vi "VIH HelpGen - Write HTML File - VI.vi"(6 "Owning Palette":cluster{"Name":string, "HTML Path":path}, 8 "error in":errorcluster, 9 "HTML Path":path, 10 "VI Path":path, 11 "Project Tree":T1) -> (0 "error out":errorcluster, 3 "dup Project Tree":T1)   [LabVIEW 2014]
doc: "::: VI Helpeks :::\nCopyright (c) 2000-2026 Konstantin Shifershteyn. All rights reserved."
uses:
  _VIH Project Manager.llb/VIH Project Tree Typedef - Tree Refnum.ctl
panel:
  # "VI Helpeks\nCopyright (c) 2012-2026 Konstantin Shifershteyn"
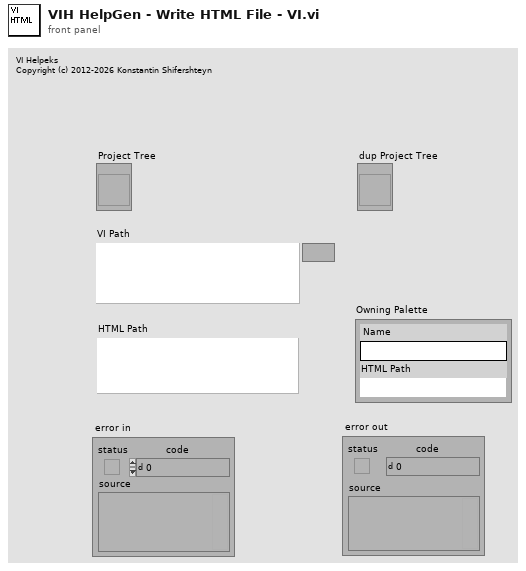
[diagram p1: front panel]
types:
  T1 = typedef "VIH Project Tree Typedef - Tree Refnum.ctl" = refnum<vi>
  T2 = typedef "VIH HelpGen Typedef - Cluster - File Rule.ctl" = cluster{"OutName":string, "BuildHelp":T3, "Source Paths":T4, "Target Paths":T5, "DscrMode":T6, "Description":string, "Control Rules":T7[], "Flags":T9, "Ctl_DscrMode":T6, "Ctl_ClustMembers":T3, "Ctl_EnumValues":T3, "MenuItemIcons":T3, "%Comments":string, "DetailsMode":T6, "DetailsText":string, "ProductInfoMode":T3, "ProductInfoText":string}
  T3 = typedef "VIH HelpGen Typedef - Enum - Default,Enable,Disable.ctl" = enum16{"Default", "Enable", "Disable"}
  T4 = typedef "VIH HelpGen Typedef - Cluster - File Rule - Source Paths.ctl" = cluster{"CSS Files":path[], "JS Files":path[], "Html Template":path}
  T5 = typedef "VIH HelpGen Typedef - Cluster - File Rule - Target Paths.ctl" = cluster{"HTML Dir":path, "Image Dir":path, "CSS Dir":path, "JS Dir":path}
  T6 = typedef "VIH HelpGen Typedef - Enum - Description Mode.ctl" = enum16{"Default", "Description", "Description1", "Description2", "Custom", "None"}
  T7 = typedef "VIH HelpGen Typedef - Cluster - Control Rule.ctl" = cluster{"CtrlID":string, "CustomRule":bool, "DscrMode":T6, "Description":string, "ClusterMembers":T3, "EnumValues":T3, "EnumValDscr":T8[], "CustomName":string}
  T8 = typedef "VIH HelpGen Typedef - Cluster - Enum Value Info.ctl" = cluster{"Value":ext, "String":string, "Description":string}
  T9 = typedef "VIH HelpGen Typedef - Cluster - Group Rule - Flags.ctl" = cluster{"Override CSS Files":bool, "Override JS Files":bool, "Override Ctl Rules":bool}
  T10 = typedef "imagedata.ctl" = cluster{"image type":i32, "image depth":i32, "image":u8[], "mask":u8[], "colors":u32[], "Rectangle":cluster{"left":i16, "top":i16, "right":i16, "bottom":i16}}
  T11 = cluster{"Original VI Name":string, "Conpane Image":T10}
  T12 = cluster{"ProductInfoMode":T3, "ProductInfoText":string}
  T13 = typedef "VIH HelpGen Typedef - Table Templates Cluster - VI Help.ctl" = cluster{"Ctrl Dscr":string, "Ring Val Dscr":string, "Enum Val Dscr":string, "VI Details":string}
  T14 = cluster{"directory path out":path, "directory path out":path, "name":string}
  T15 = cluster{string[], "Control Rules":T7[], "Ctl_DscrMode":T6, "Ctl_ClustMembers":T3, "Ctl_EnumValues":T3}
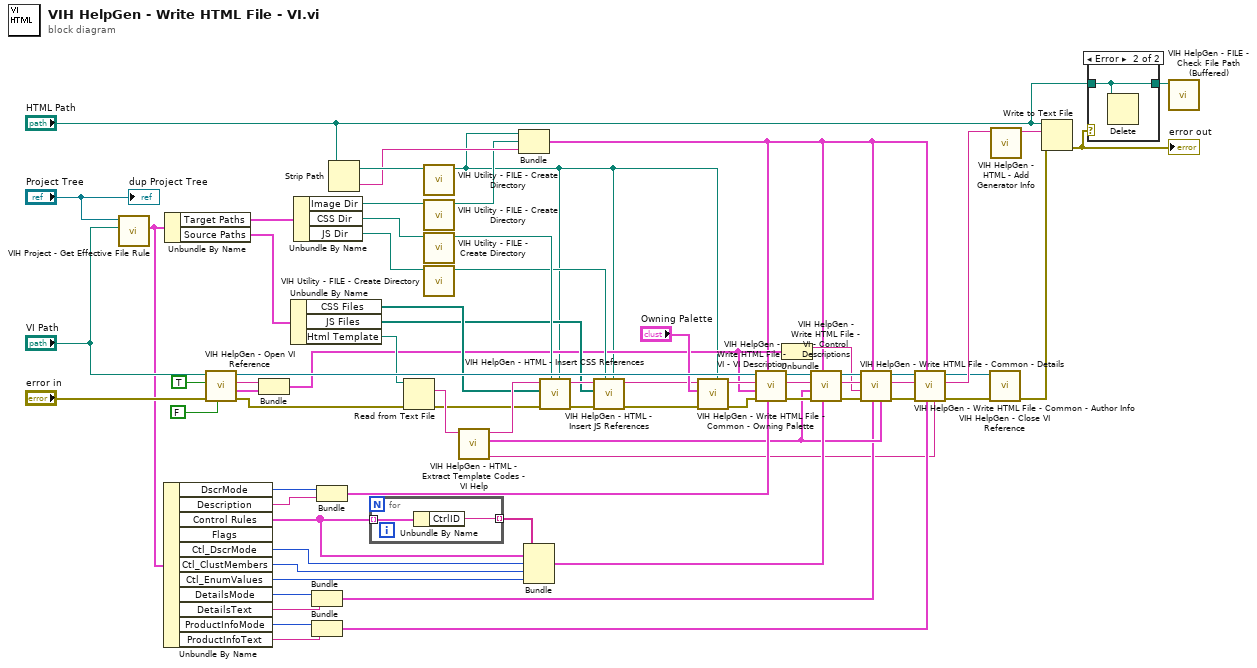
[diagram p0: block diagram]
diagram:
  n1 = call "VIH Project - Get Effective File Rule.vi"("File Path"="VI Path", "Project Tree"="Project Tree") -> ("Effective File Rule"=w48:T2)  [unwired: 6 in, 3 out]
  n2 = Unbundle By Name(w48) -> ("DscrMode"=w47:T6, "Description"=w46:string, "Control Rules"=w41:T7[], "Ctl_DscrMode"=w44:T6, "Ctl_ClustMembers"=w43:T3, "Ctl_EnumValues"=w42:T3, "DetailsMode"=w27:T6, "DetailsText"=w26:string, "ProductInfoMode"=w9:T3, "ProductInfoText"=w8:string)  [unwired: 1 out]
  n3 = Unbundle By Name(w48) -> ("Target Paths"=w63:T5, "Source Paths"=w62:T4)
  n4 = call "VIH HelpGen - Open VI Reference.vi"("Enable Conpane Image Check (T)"=FALSE, "error in"="error in", "Force use wrapper (F)"=TRUE, "VI Path"="VI Path") -> ("error out"=w59:errorcluster, "Conpane Image"=w22:T10, "Original VI Name"=w23:string, "VI Reference"=w65:refnum<vi>)  [unwired: 4 in]
  n5 = Bundle("Original VI Name"=w23, "Conpane Image"=w22) -> (w21:T11)  [unwired: 1 in]
  n6 = Unbundle By Name(w62) -> ("CSS Files"=w61:path[], "JS Files"=w32:path[], "Html Template"=w60:path)
  n7 = Unbundle By Name(w63) -> ("Image Dir"=w49:path, "CSS Dir"=w51:path, "JS Dir"=w38:path)
  n8 = Bundle("DetailsMode"=w27, "DetailsText"=w26) -> (w24:cluster{"DetailsMode":T6, "DetailsText":string})  [unwired: 1 in]
  n9 = Bundle("ProductInfoMode"=w9, "ProductInfoText"=w8) -> (w7:T12)  [unwired: 1 in]
  n10 = Bundle("DscrMode"=w47, "Description"=w46) -> (w45:cluster{"DscrMode":T6, "Description":string})  [unwired: 1 in]
  n11 = Strip Path(path="HTML Path") -> (stripped path=w52:path, name=w4:string)
  n12 = for {
    tunnel: w41 -> [w73] mode=indexing
    tunnel: [w72] -> w40 mode=indexing
    n13 = Unbundle By Name(w73) -> ("CtrlID"=w72:string)
  }
  n14 = Read from Text File(file (use dialog)=w60, error in=w59) -> (text=w67:string, error out=w58:errorcluster)  [unwired: 2 in, 2 out]
  n15 = call "VIH Utility - FILE - Create Directory.vi"("directory path"=w52) -> ("directory path out"=w1:path)  [unwired: 6 in, 2 out]
  n16 = call "VIH Utility - FILE - Create Directory.vi"("directory path"=w49) -> ("directory path out"=w3:path)  [unwired: 6 in, 2 out]
  n17 = call "VIH Utility - FILE - Create Directory.vi"("directory path"=w51) -> ("directory path out"=w50:path)  [unwired: 6 in, 2 out]
  n18 = call "VIH Utility - FILE - Create Directory.vi"("directory path"=w38) -> ("directory path out"=w33:path)  [unwired: 6 in, 2 out]
  n19 = call "VIH HelpGen - HTML - Extract Template Codes - VI Help.vi"("HTML in"=w67) -> ("ProductInfo Template"=w6:string, "Table Templates"=w25:T13, "HTML out"=w64:string)  [unwired: 8 in]
  n20 = Bundle("directory path out"=w1, "directory path out"=w3, "name"=w4) -> (w2:T14)  [unwired: 1 in]
  n21 = Bundle(w40, "Control Rules"=w41, "Ctl_DscrMode"=w44, "Ctl_ClustMembers"=w43, "Ctl_EnumValues"=w42) -> (w39:T15)  [unwired: 1 in]
  n22 = call "VIH HelpGen - HTML - Insert CSS References.vi"("HTML Folder"=w1, "CSS Folder"=w50, "error in"=w58, "CSS files"=w61, "HTML in"=w64) -> ("error out"=w36:errorcluster, "HTML out"=w37:string)  [unwired: 5 in]
  n23 = call "VIH HelpGen - HTML - Insert JS References.vi"("HTML Folder"=w1, "JSS Folder"=w33, "error in"=w36, "JS files"=w32, "HTML in"=w37) -> ("error out"=w35:errorcluster, "HTML out"=w34:string)  [unwired: 5 in]
  n24 = call "VIH HelpGen - Write HTML File - Common - Owning Palette.vi"("HTML Folder"=w1, "error in"=w35, "Owning Palette"="Owning Palette", "HTML in"=w34) -> ("error out"=w56:errorcluster, "HTML out"=w57:string)  [unwired: 6 in]
  n25 = call "VIH HelpGen - Write HTML File - VI - VI Description.vi"("Description Params"=w45, "Save params"=w2, "error in"=w56, "Original VI Info"=w21, "HTML in"=w57, "VI Reference"=w65) -> ("error out"=w69:errorcluster, "HTML out"=w68:string, "dup VI Reference"=w70:refnum<vi>)  [unwired: 3 in]
  n26 = Unbundle(w21) -> ("Original VI Name"=w20:string)  [unwired: 1 out]
  n27 = call "VIH HelpGen - Write HTML File - VI - Control Descriptions.vi"("Ctrl Dscr Params"=w39, "Save params"=w2, "error in"=w69, "Table Templates"=w25, "HTML in"=w68, "VI Reference"=w70) -> ("error out"=w28:errorcluster, "HTML out"=w29:string, "dup VI Reference"=w30:refnum<vi>)  [unwired: 3 in]
  n28 = call "VIH HelpGen - Write HTML File - Common - Details.vi"("Templates"=w25, "Details Params"=w24, "Save params"=w2, "error in"=w28, "Original VI Name"=w20, "HTML in"=w29, "VI Reference"=w30) -> ("error out"=w14:errorcluster, "HTML out"=w13:string, "dup VI Reference"=w15:refnum<vi>)  [unwired: 2 in]
  n29 = call "VIH HelpGen - Write HTML File - Common - Author Info.vi"("Product Info Template"=w6, "Product Info"=w7, "Save params"=w2, "error in"=w14, "HTML in"=w13, "VI Reference"=w15) -> ("error out"=w10:errorcluster, "HTML out"=w12:string, "dup VI Reference"=w11:refnum<vi>)  [unwired: 3 in]
  n30 = call "VIH HelpGen - Close VI Reference.vi"("error in"=w10, "VI Reference"=w11) -> ("error out"=w66:errorcluster)  [unwired: 9 in]
  n31 = call "VIH HelpGen - HTML - Add Generator Info.vi"("HTML in"=w12) -> ("HTML out"=w16:string)  [unwired: 10 in]
  n32 = Write to Text File(file (use dialog)="HTML Path", text=w16, error in=w66) -> (error out=w18:errorcluster)  [unwired: 1 in, 2 out]
  "error out" <- w18
  n33 = case shown="Error" w18 {
    tunnel: "HTML Path" -> [w74 w75]
    tunnel: [w74 w75] -> w19
    frame No Error {
    }
    frame Error {
      n34 = Delete(path (use dialog)=w75) -> ()  [unwired: 4 in, 3 out]
    }
  }
  n35 = call "VIH HelpGen - FILE - Check File Path (Buffered).vi"("File Path"=w19) -> ()  [unwired: 9 in, 2 out]
  "dup Project Tree" <- "Project Tree"
